vi "sync start of cycle.vi"(8 "error in (no error)":errorcluster, 10 "parameters data in":T1, 11 "module in":refnum<class "Shared Memory runtime.lvclass">) -> (0 "error out":errorcluster, 2 "parameters data out":T1, 3 "module out":refnum<class "Shared Memory runtime.lvclass">)   [LabVIEW 2014, in "Shared Memory runtime.lvclass"]
uses:
  Shared Memory runtime.lvclass
  <vilib>/NI/Tag Bus/table/data table.ctl
  Shared Memory runtime.lvclass/Shared Memory runtime.ctl
  <vilib>/NI/NI Linux RT IPC/POSIX Threads/Classes/Semaphore/Public VIs/Semaphore Post.vi
  <vilib>/NI/NI Linux RT IPC/POSIX Threads/Classes/Semaphore/Public VIs/Semaphore Get Value.vi
  <vilib>/NI/NI Linux RT IPC/POSIX Threads/Classes/Semaphore/Semaphore.lvclass
  <vilib>/NI/NI Linux RT IPC/Shared Memory/Classes/Shared Memory/Shared Memory.lvclass
  <vilib>/NI/Tag Bus/table/data table.lvlib
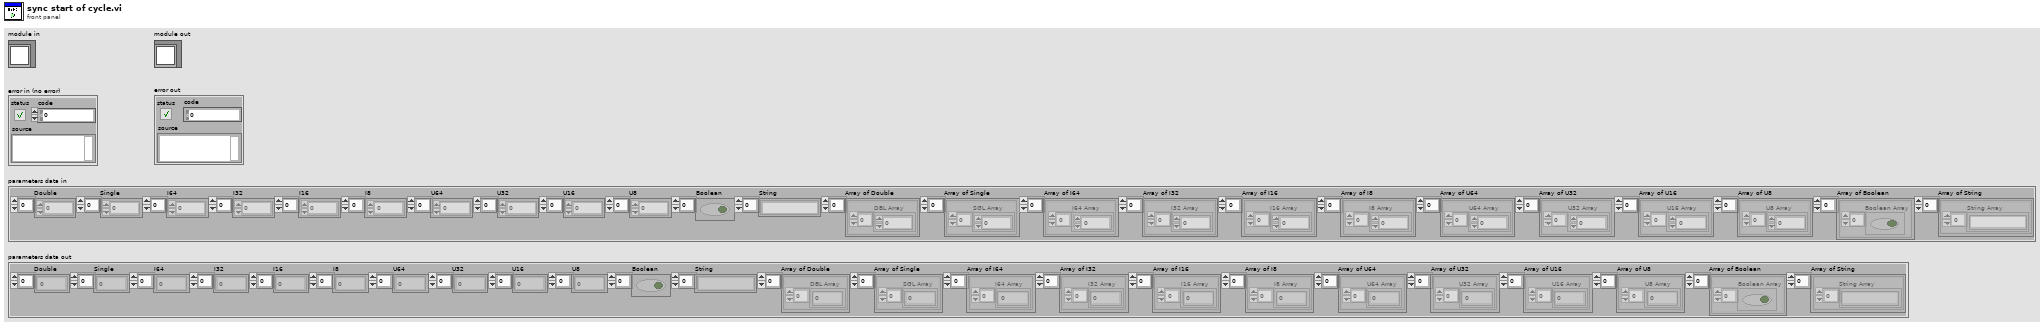
[diagram p1: front panel]
types:
  T1 = typedef "tag bus.lvlib/data table.lvlib/data table.ctl" = cluster{"Double":dbl[], "Single":sgl[], "I64":i64[], "I32":i32[], "I16":i16[], "I8":i8[], "U64":u64[], "U32":u32[], "U16":u16[], "U8":u8[], "Boolean":bool[], "String":string[], "Array of Double":cluster{"DBL Array":dbl[]}[], "Array of Single":cluster{"SGL Array":sgl[]}[], "Array of I64":cluster{"I64 Array":i64[]}[], "Array of I32":cluster{"I32 Array":i32[]}[], "Array of I16":cluster{"I16 Array":i16[]}[], "Array of I8":cluster{"I8 Array":i8[]}[], "Array of U64":cluster{"U64 Array":u64[]}[], "Array of U32":cluster{"U32 Array":u32[]}[], "Array of U16":cluster{"U16 Array":u16[]}[], "Array of U8":cluster{"U8 Array":u8[]}[], "Array of Boolean":cluster{"Boolean Array":bool[]}[], "Array of String":cluster{"String Array":string[]}[]}
  T2 = typedef "Shared Memory runtime.lvclass/sync data.ctl" = cluster{"semaphores soc":T3[], "semaphores eoc":T3[], "timeout":dbl, "enabled":bool, "sync shared memory":T5, "publish timing":bool, "timing indices":T6, "timing pointers":T7}
  T3 = typedef "Shared Memory runtime.lvclass/semaphore data.ctl" = cluster{"semaphore":T4, "name":string}
  T4 = typedef "Linux RT IPC.POSIX Threads.lvlib/Semaphore.lvclass/reference.ctl" = refnum<data-value>
  T5 = typedef "Linux RT IPC.Shared Memory.lvlib/reference.ctl" = refnum<data-value>
  T6 = typedef "Shared Memory runtime.lvclass/sync timing indices.ctl" = cluster{"start time index":i32}
  T7 = typedef "Shared Memory runtime.lvclass/sync timing pointers.ctl" = cluster{"start sec ptr":u64, "start nsec ptr":u64}
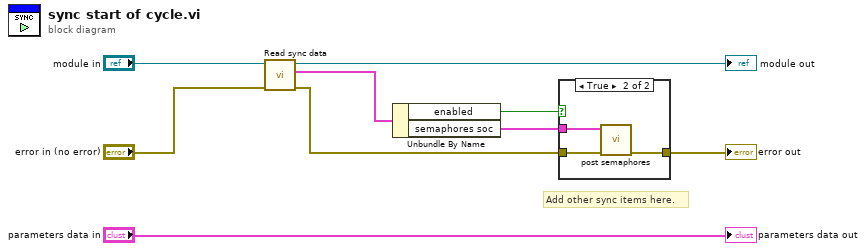
[diagram p0: block diagram]
diagram:
  # "Add other sync items here."
  n1 = call "Read sync data.vi"("error in (no error)"="error in (no error)", "Shared Memory runtime in"="module in") -> ("error out"=w3:errorcluster, "sync data"=w1:T2, "Shared Memory runtime out"=→"module out":refnum<class "Shared Memory runtime.lvclass">)  [unwired: 7 in]
  n2 = Unbundle By Name(w1) -> ("enabled"=w7:bool, "semaphores soc"=w9:T3[])
  n3 = case shown="True" w7 {
    tunnel: w3 -> [w10 w13]
    tunnel: w9 -> [_ w12]
    tunnel: [w10 w11] -> w8
    frame False {
    }
    frame True {
      n4 = call "post semaphores.vi"("error in (no error)"=w13, "semaphores in"=w12) -> ("error out"=w11:errorcluster)  [unwired: 8 in, 1 out]
    }
  }
  "error out" <- w8
  "parameters data out" <- "parameters data in"
